vi "Model Cleanup Done.vi"(11 "IModel in":refnum<class "IModel.lvclass">) -> (3 "IModel out":refnum<class "IModel.lvclass">)   [LabVIEW 2018, in "MVA Framework.lvlib" / "IModel.lvlib" / "IModel.lvclass"]
doc: "模型清理完成"
uses:
  IModel.lvclass
  <vilib>/ActorFramework/Message Enqueuer/Message Enqueuer.lvclass
  <vilib>/ActorFramework/Message/Message.lvclass
  <vilib>/ActorFramework/Actor/Actor.lvclass
  IObserver/IObserver/IObserver.lvclass
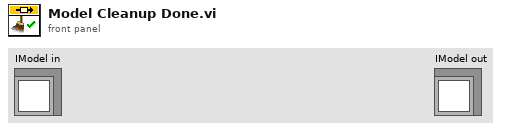
[diagram p1: front panel]
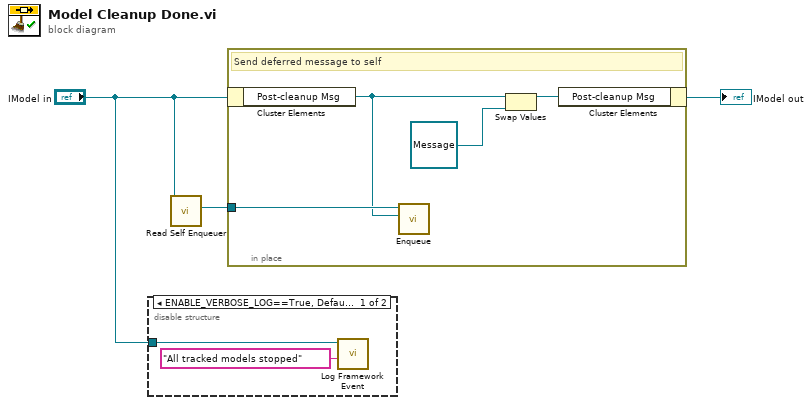
[diagram p0: block diagram]
diagram:
  n1 = disable-structure shown="ENABLE_VERBOSE_LOG==True, Default" {
    disable-tunnel: "IModel in" -> [w4 _]
    frame condition #0 (active) {
      # "Log end-of-shutdown event"
      n2 = call "Log Framework Event.vi"("Data To Log"="All tracked models stopped" ("Description"), "IObserver in"=w4) -> ()  [unwired: 9 in, 1 out]
    }
    frame condition #1 {
      # "Remove logging at compile time"
    }
  }
  n3 = call <vilib>:"Read Self Enqueuer.vi"("Actor"="IModel in") -> ("Self Enqueuer"=w3:refnum<class "Message Enqueuer.lvclass">)  [unwired: 10 in]
  n4 = in-place {
    in-place-border: w3 -> [w9]
    # "Send deferred message to self"
    n5 = in-place-cluster #1("IModel in") -> ("Post-cleanup Msg"=w8:refnum<class "Message.lvclass">)
    n6 = call <vilib>:"Enqueue.vi"("Message"=w8, "Message Enqueuer in"=w9) -> ()  [unwired: 8 in, 2 out]
    n7 = Swap Values(12:w8, 14:refnum<class "Message.lvclass"> refnum ("Final Last Ack Message")) -> (1:w7:refnum<class "Message.lvclass">)  [unwired: 1 in, 1 out]
    n8 = in-place-cluster #1("Post-cleanup Msg"=w7) -> (→"IModel out":refnum<class "IModel.lvclass">)
  }
